vi "Periodic Tasks.vi"(8 "error in":errorcluster) -> ()   [LabVIEW 2018]
doc: "This VI runs in parallel to other tasks. It can contain as many user-defined periodic loops as you need. These can carry out PID or other sorts of timed response."
uses:
  <vilib>/Rock Robotics/WPI/Solenoid/WPI_SolenoidValue.ctl
  <vilib>/Rock Robotics/WPI/ThirdParty/Phoenix-LabVIEW/Motor Controller/Controls/CTRE_Phoenix_MotorControl_ControlMode.ctl
  <vilib>/Rock Robotics/WPI/Utilities/WPI_GetSetVariantRefNum.vi
  <vilib>/Rock Robotics/WPI/Solenoid/WPI_SolenoidSetEnum.vi
  Global 1.vi
  <vilib>/Rock Robotics/Network Tables/NT Write Boolean.vi
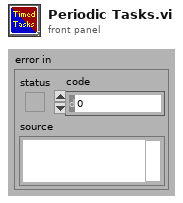
[diagram p1: front panel]
types:
  T1 = typedef "WPI_JoystickDevRef.ctl" = cluster{"Device":T2}
  T2 = typedef "WPI_JoystickDeviceEnum.ctl" = enum16{"USB 0", "USB 1", "USB 2", "USB 3", "USB 4", "USB 5"}
  T3 = typedef "WPI_RobotDriveDevRef.ctl" = cluster{"DevStatus":errorcluster, "Motors[]":T4[], "Square Inputs":bool, "Max Output":dbl}
  T4 = typedef "WPI_MotorControlDeviceRef.ctl" = cluster{"DeviceStatus":errorcluster, "Type":T5, "PWM":cluster{"PWM Channel":T6, "DeadBand":T7}, "CAN":cluster{"Device Number":u8, "SetOutput VI Ref":variant, "GetOutput VI Ref":variant, "Enable VI Ref":variant, "Disable VI Ref":variant, "Data":variant}, "Invert":bool, "DIO PWM":cluster{"PWM \"Enable\" Channel":T6, "DIOChannel":T8, "PWM Rate":dbl}}
  T5 = typedef "WPI_MotorControlType.ctl" = enum16{"PWM", "CAN", "DIO PWM"}
  T6 = typedef "FPGA_DIOPWMChannel.ctl" = enum8{"PWM 0", "PWM 1", "PWM 2", "PWM 3", "PWM 4", "PWM 5", "PWM 6", "PWM 7", "PWM 8", "PWM 9", "PWM MXP 0", "PWM MXP 1", "PWM MXP 2", "PWM MXP 3", "PWM MXP 4", "PWM MXP 5", "PWM MXP 6", "PWM MXP 7", "PWM MXP 8", "PWM MXP 9", "Invalid"}
  T7 = typedef "WPI_PWMDeadband.ctl" = cluster{"Name":string, "maxPositivePwm":i32, "minPositivePwm":i32, "centerPwm":i32, "maxNegativePwm":i32, "minNegativePwm":i32, "angularRange":u16}
  T8 = typedef "FPGA_DIOChannel.ctl" = enum8{"DIO 0", "DIO 1", "DIO 2", "DIO 3", "DIO 4", "DIO 5", "DIO 6", "DIO 7", "DIO 8", "DIO 9", "DIO MXP 0", "DIO MXP 1", "DIO MXP 2", "DIO MXP 3", "DIO MXP 4", "DIO MXP 5", "DIO MXP 6", "DIO MXP 7", "DIO MXP 8", "DIO MXP 9", "DIO MXP 10", "DIO MXP 11", "DIO MXP 12", "DIO MXP 13", "DIO MXP 14", "DIO MXP 15", "SPI Port CS1", "SPI Port CS2", "SPI Port CS3", "SPI Port MISO", "SPI Port MOSI", "Invalid"}
  T9 = cluster{"JoystickDevRef":T1, "RobotDriveDevRef":T3}
  T10 = typedef "WPI_SolenoidDevRef.ctl" = cluster{"DevStatus":errorcluster, "Pneumatics Control Module":u8, "Forward Solenoid Channel":T11, "Reverse Solenoid Channel":T11}
  T11 = typedef "WPI_SolenoidChannel.ctl" = enum8{"Solenoid 0", "Solenoid 1", "Solenoid 2", "Solenoid 3", "Solenoid 4", "Solenoid 5", "Solenoid 6", "Solenoid 7", "Invalid"}
  T12 = typedef "WPI_SolenoidValue.ctl" = enum16{"Off", "On", "Forward", "Reverse"}
  T13 = typedef "WPI_SwitchDevRef.ctl" = cluster{"DevStatus":errorcluster, "DIO Channel":T8, "CntIndex":T14, "Normally Closed":bool}
  T14 = typedef "FPGA_CounterCtrSystemIndex.ctl" = enum8{"Ctr 0", "Ctr 1", "Ctr 2", "Ctr 3", "Ctr 4", "Ctr 5", "Ctr 6", "Ctr 7", "Invalid"}
  T15 = typedef "WPI_EncoderDevRef.ctl" = cluster{"DevStatus":errorcluster, "EncoderIndex":T16, "CounterIndex":T14, "DistancePerCount":dbl, "Decoding Type":T17}
  T16 = typedef "FPGA_EncoderIdx.ctl" = enum8{"Enc 0", "Enc 1", "Enc 2", "Enc 3", "Enc 4", "Enc 5", "Enc 6", "Enc 7", "Invalid"}
  T17 = typedef "WPI_EncoderType.ctl" = enum16{"1x", "2x", "4x"}
  T18 = typedef "CTRE_Phoenix_MotorControl_ControlMode.ctl" = u16
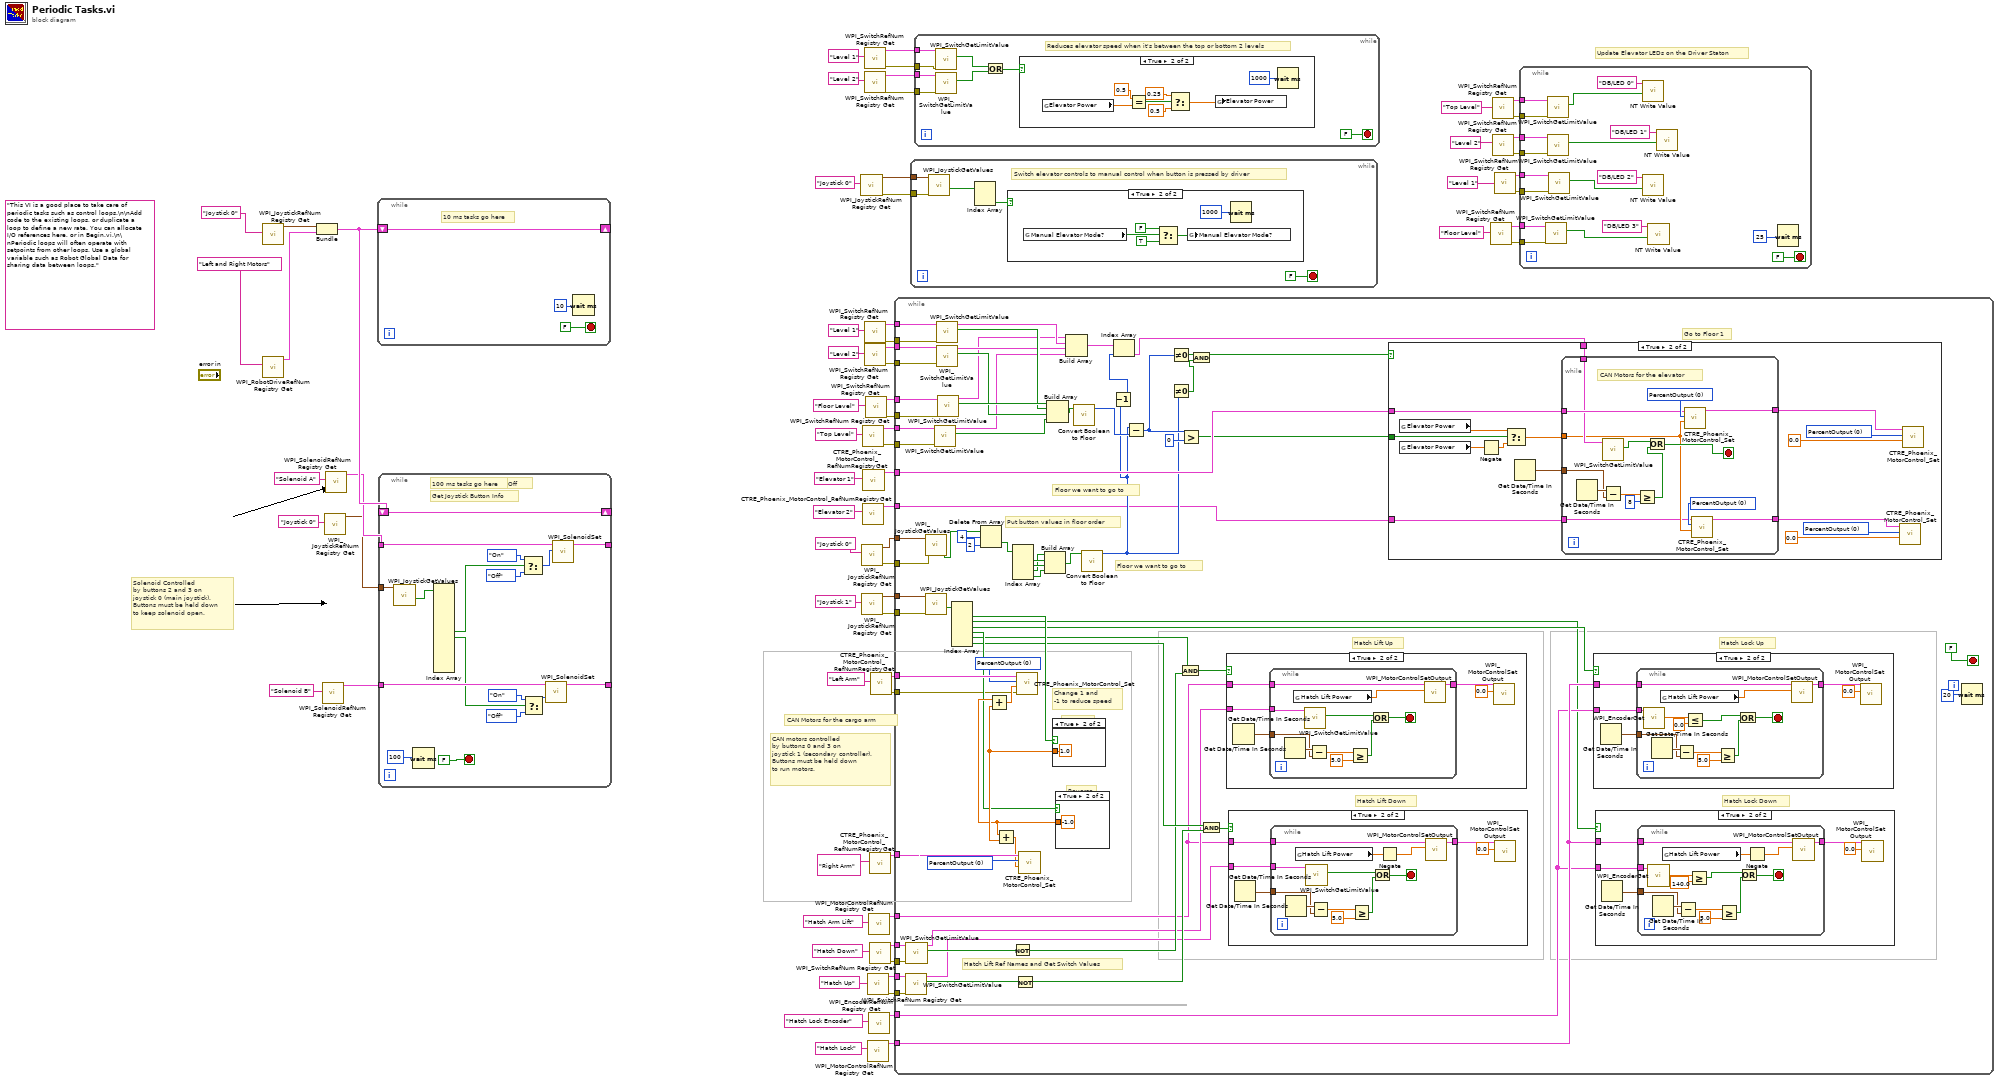
[diagram p0: block diagram]
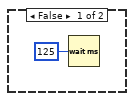
[diagram p2: hidden frame]
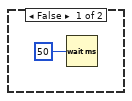
[diagram p3: hidden frame]
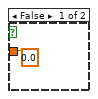
[diagram p9: hidden frame]
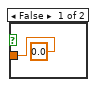
[diagram p10: hidden frame]
diagram:
  (unwired) "This VI is a good place to take care of periodic tasks such as control loops.\n\nAdd code to the existing loops, or duplicate a loop to define a new rate. You can allocate I/O references here, or in Begin.vi.\n\nPeriodic loops will often operate with setpoints from other loops. Use a global variable such as Robot Global Data for sharing data between loops."
  # "Update Elevator LEDs on the Driver Staton"
  # "CAN Motors for the cargo arm"
  # "CAN motors controlled\nby buttons 0 and 3 on \njoystick 1 (secondary controller).\nButtons must be held down\nto run motors."
  # "Solenoid Controlled\nby buttons 2 and 3 on \njoystick 0 (main joystick).\nButtons must be held down\nto keep solenoid open."
  n1 = call <vilib>:"WPI_JoystickRefNum Registry Get.vi"("refnum name"="Joystick 0") -> ("JoystickDevRef"=w69:T1)  [unwired: 1 in, 9 out]
  n2 = call <vilib>:"WPI_RobotDriveRefNum Registry Get.vi"("refnum name"="Left and Right Motors") -> ("RobotDriveDevRef"=w68:T3)  [unwired: 1 in, 9 out]
  n3 = Bundle("JoystickDevRef"=w69, "RobotDriveDevRef"=w68) -> (w67:T9)  [unwired: 1 out]
  n4 = call <vilib>:"WPI_SolenoidRefNum Registry Get.vi"("refnum name"="Solenoid B") -> ("SolenoidDevRef"=w62:T10)  [unwired: 9 in, 1 out]
  n5 = call <vilib>:"WPI_JoystickRefNum Registry Get.vi"("refnum name"="Joystick 0") -> ("JoystickDevRef"=w59:T1)  [unwired: 9 in, 1 out]
  n6 = call <vilib>:"WPI_SolenoidRefNum Registry Get.vi"("refnum name"="Solenoid A") -> ("SolenoidDevRef"=w63:T10)  [unwired: 9 in, 1 out]
  n7 = while {
    shift-right: [w72] -> _
    shift-left: w67 -> [w72]
    stop <- FALSE stop-if-true
    # "10 ms tasks go here"
    n8 = Wait (ms)(milliseconds to wait=u32 10) -> ()  [unwired: 1 out]
  }
  n9 = while {
    shift-right: [w89] -> _
    shift-left: w67 -> [w89]
    tunnel: w63 -> [w82]
    tunnel: w62 -> [w81]
    tunnel: [w80] -> _
    tunnel: [w79] -> _
    tunnel: w59 -> [w78]
    stop <- FALSE stop-if-true
    # "Get Joystick Button Info"
    # "Turn the solenoid On or Off"
    # "100 ms tasks go here"
    n10 = call <vilib>:"WPI_JoystickGetValues.vi"("JoystickDevRef"=w78) -> ("Buttons"=w77:bool[])  [unwired: 6 in, 4 out]
    n11 = Wait (ms)(milliseconds to wait=u32 100) -> ()  [unwired: 1 out]
    n12 = Index Array(array=w77) -> (element #7=w76:bool, element #8=w75:bool)  [unwired: 14 in, 12 out]
    n13 = Select(t=WPI_SolenoidValue."On" ("Value"), s=w76, f=WPI_SolenoidValue."Off" ("Value")) -> (s? t:f=w86:T12)
    n14 = Select(t=WPI_SolenoidValue."On" ("Value"), s=w75, f=WPI_SolenoidValue."Off" ("Value")) -> (s? t:f=w83:T12)
    n15 = call-poly <vilib>:"WPI_SolenoidSet.vi"("Value"=w83, "SolenoidDevRef"=w81) -> ("SolenoidDevRef"=w79:T10)  [unwired: 1 in, 8 out]
    n16 = call-poly <vilib>:"WPI_SolenoidSet.vi"("Value"=w86, "SolenoidDevRef"=w82) -> ("SolenoidDevRef"=w80:T10)  [unwired: 1 in, 8 out]
  }
  n17 = call <vilib>:"WPI_JoystickRefNum Registry Get.vi"("refnum name"="Joystick 0") -> ("error out"=w46:errorcluster, "JoystickDevRef"=w47:T1)  [unwired: 9 in]
  n18 = call <vilib>:"WPI_JoystickRefNum Registry Get.vi"("refnum name"="Joystick 0") -> ("error out"=w40:errorcluster, "JoystickDevRef"=w53:T1)  [unwired: 9 in]
  n19 = call <vilib>:"WPI_JoystickRefNum Registry Get.vi"("refnum name"="Joystick 1") -> ("error out"=w45:errorcluster, "JoystickDevRef"=w55:T1)  [unwired: 9 in]
  n20 = call <vilib>:"WPI_SwitchRefNum Registry Get.vi"("refnum name"="Top Level") -> ("error out"=w44:errorcluster, "SwitchDevRef"=w56:T13)  [unwired: 9 in]
  n21 = call <vilib>:"CTRE_Phoenix_MotorControl_RefNumRegistryGet.vi"("refnum name"="Elevator 2") -> ("PhoenixMotorControlDevRef"=w7:T4)  [unwired: 9 in, 1 out]
  n22 = call <vilib>:"CTRE_Phoenix_MotorControl_RefNumRegistryGet.vi"("refnum name"="Elevator 1") -> ("PhoenixMotorControlDevRef"=w54:T4)  [unwired: 9 in, 1 out]
  n23 = call <vilib>:"WPI_SwitchRefNum Registry Get.vi"("refnum name"="Level 1") -> ("error out"=w1:errorcluster, "SwitchDevRef"=w4:T13)  [unwired: 9 in]
  n24 = call <vilib>:"WPI_SwitchRefNum Registry Get.vi"("refnum name"="Level 2") -> ("error out"=w2:errorcluster, "SwitchDevRef"=w3:T13)  [unwired: 9 in]
  n25 = call <vilib>:"WPI_SwitchRefNum Registry Get.vi"("refnum name"="Level 1") -> ("error out"=w41:errorcluster, "SwitchDevRef"=w66:T13)  [unwired: 9 in]
  n26 = call <vilib>:"WPI_SwitchRefNum Registry Get.vi"("refnum name"="Level 2") -> ("error out"=w42:errorcluster, "SwitchDevRef"=w65:T13)  [unwired: 9 in]
  n27 = call <vilib>:"WPI_SwitchRefNum Registry Get.vi"("refnum name"="Floor Level") -> ("error out"=w43:errorcluster, "SwitchDevRef"=w52:T13)  [unwired: 9 in]
  n28 = call <vilib>:"WPI_SwitchRefNum Registry Get.vi"("refnum name"="Hatch Up") -> ("error out"=w22:errorcluster, "SwitchDevRef"=w23:T13)  [unwired: 9 in]
  n29 = call <vilib>:"WPI_MotorControlRefNum Registry Get.vi"("refnum name"="Hatch Lock") -> ("MotorControlDevRef"=w17:T4)  [unwired: 9 in, 1 out]
  n30 = call <vilib>:"WPI_MotorControlRefNum Registry Get.vi"("refnum name"="Hatch Arm Lift") -> ("MotorControlDevRef"=w19:T4)  [unwired: 9 in, 1 out]
  n31 = call <vilib>:"WPI_EncoderRefNum Registry Get.vi"("refnum name"="Hatch Lock Encoder") -> ("EncoderDevRef"=w18:T15)  [unwired: 9 in, 1 out]
  n32 = call <vilib>:"WPI_SwitchRefNum Registry Get.vi"("refnum name"="Hatch Down") -> ("error out"=w21:errorcluster, "SwitchDevRef"=w20:T13)  [unwired: 9 in]
  n33 = call <vilib>:"CTRE_Phoenix_MotorControl_RefNumRegistryGet.vi"("refnum name"="Right Arm") -> ("PhoenixMotorControlDevRef"=w57:T4)  [unwired: 9 in, 1 out]
  n34 = call <vilib>:"CTRE_Phoenix_MotorControl_RefNumRegistryGet.vi"("refnum name"="Left Arm") -> ("error out"=w39:errorcluster, "PhoenixMotorControlDevRef"=w58:T4)  [unwired: 9 in]
  n35 = while {
    tunnel: w66 -> [w165]
    tunnel: w65 -> [w164]
    tunnel: w58 -> [w163]
    tunnel: w57 -> [w162]
    tunnel: w56 -> [w161]
    tunnel: w55 -> [w160]
    tunnel: w54 -> [w157]
    tunnel: w53 -> [w159]
    tunnel: w52 -> [w158]
    tunnel: w45 -> [w147]
    tunnel: w44 -> [w146]
    tunnel: w43 -> [w145]
    tunnel: w42 -> [w144]
    tunnel: w41 -> [w143]
    tunnel: w40 -> [w142]
    tunnel: w39 -> [w141]
    tunnel: w23 -> [w140]
    tunnel: w22 -> [w139]
    tunnel: w21 -> [w138]
    tunnel: w20 -> [w137]
    tunnel: w19 -> [w127]
    tunnel: w18 -> [w124]
    tunnel: w17 -> [w125]
    tunnel: w7 -> [w92]
    stop <- FALSE stop-if-true
    w154 = T18 0 items=["PercentOutput"=0, "Position"=1, "Velocity"=2, "Current"=3, "Follower"=5, "MotionProfile"=6, "MotionMagic"=7, "MotionProfileArc"=10, "Disabled"=15] ("Control Mode")
    w156 = T18 0 items=["PercentOutput"=0, "Position"=1, "Velocity"=2, "Current"=3, "Follower"=5, "MotionProfile"=6, "MotionMagic"=7, "MotionProfileArc"=10, "Disabled"=15] ("Control Mode")
    # "Put button values in floor order"
    # "Floor we want to go to"
    # "Floor we want to go to"
    # "Go to Floor 1"
    # "Hatch Lock Down"
    # "Hatch Lock Up"
    # "Hatch Lift Ref Names and Get Switch Values"
    # "Hatch Lift Down"
    # "Hatch Lift Up"
    # "Change 1 and\n-1 to reduce speed"
    # "Forward"
    # "Reverse"
    n36 = call <vilib>:"WPI_SwitchGetLimitValue.vi"("error in (no error)"=w139, "SwitchDevRef"=w140) -> ("Switch Pressed"=w134:bool, "SwitchDevRef"=w126:T13)  [unwired: 7 in, 1 out]
    n37 = call <vilib>:"WPI_SwitchGetLimitValue.vi"("error in (no error)"=w138, "SwitchDevRef"=w137) -> ("Switch Pressed"=w132:bool, "SwitchDevRef"=w128:T13)  [unwired: 7 in, 1 out]
    n38 = call <vilib>:"WPI_JoystickGetValues.vi"("error in (no error)"=w142, "JoystickDevRef"=w159) -> ("Buttons"=w93:bool[])  [unwired: 5 in, 4 out]
    n39 = call <vilib>:"WPI_JoystickGetValues.vi"("error in (no error)"=w147, "JoystickDevRef"=w160) -> ("Buttons"=w151:bool[])  [unwired: 5 in, 4 out]
    n40 = call <vilib>:"WPI_SwitchGetLimitValue.vi"("error in (no error)"=w146, "SwitchDevRef"=w161) -> ("Switch Pressed"=w118:bool, "SwitchDevRef"=w101:T13)  [unwired: 7 in, 1 out]
    n41 = call <vilib>:"WPI_SwitchGetLimitValue.vi"("error in (no error)"=w143, "SwitchDevRef"=w165) -> ("Switch Pressed"=w110:bool, "SwitchDevRef"=w103:T13)  [unwired: 7 in, 1 out]
    n42 = call <vilib>:"WPI_SwitchGetLimitValue.vi"("error in (no error)"=w144, "SwitchDevRef"=w164) -> ("Switch Pressed"=w109:bool, "SwitchDevRef"=w102:T13)  [unwired: 7 in, 1 out]
    n43 = call <vilib>:"WPI_SwitchGetLimitValue.vi"("error in (no error)"=w145, "SwitchDevRef"=w158) -> ("Switch Pressed"=w117:bool, "SwitchDevRef"=w100:T13)  [unwired: 7 in, 1 out]
    n44 = Index Array(array=w151) -> (element #1=w149:bool, element #2=w122:bool, element #3=w123:bool, element #4=w148:bool, element #5=w136:bool, element #6=w135:bool)  [unwired: 6 in]
    n45 = Delete From Array(array=w93, length=4, index=2) -> (deleted portion=w116:bool[])  [unwired: 1 out]
    n46 = Not(x=w132) -> (.not. x?=w131:bool)
    n47 = Index Array(array=w116) -> (element #1=w115:bool, element #2=w114:bool, element #3=w113:bool, element #4=w112:bool)  [unwired: 4 in]
    n48 = Not(x=w134) -> (.not. x?=w130:bool)
    n49 = Build Array(w113, w115, w114, w112) -> (w111:bool[])
    n50 = Build Array(w117, w110, w109, w118) -> (w119:bool[])
    n51 = case shown="True" w149 {
      tunnel: [0.0 1.0] -> w152
      frame False {
      }
      frame True {
      }
    }
    n52 = case shown="True" w148 {
      tunnel: [0.0 -1.0] -> w150
      frame False {
      }
      frame True {
      }
    }
    n53 = Add(x=w150, y=w152) -> (x+y=w155:dbl)
    n54 = Add(x=w150, y=w152) -> (x+y=w153:dbl)
    n55 = call <vilib>:"CTRE_Phoenix_MotorControl_Set.vi"("error in (no error)"=w141, "Output"=w155, "Control Mode"=w156, "PhoenixMotorControlDevRef"=w163) -> ()  [unwired: 6 in, 2 out]
    n56 = call <vilib>:"CTRE_Phoenix_MotorControl_Set.vi"("Output"=w153, "Control Mode"=w154, "PhoenixMotorControlDevRef"=w162) -> ()  [unwired: 7 in, 2 out]
    n57 = Build Array(w100, w103, w102, w101) -> (w99:T13[])
    n58 = call "Convert Boolean to Floor.vi"("Boolean array"=w119) -> ("Floor Number"=w107:i32)  [unwired: 8 in, 2 out]
    n59 = call "Convert Boolean to Floor.vi"("Boolean array"=w111) -> ("Floor Number"=w95:i32)  [unwired: 8 in, 2 out]
    n60 = Decrement(x=w95) -> (x-1=w97:i32)
    n61 = Index Array(array=w99, index=w97) -> (element=w98:T13)
    n62 = Subtract(x=w95, y=w107) -> (x-y=w106:i32)
    n63 = Not Equal To 0?(x=w106) -> (x != 0?=w108:bool)
    n64 = Not Equal To 0?(x=w95) -> (x != 0?=w94:bool)
    n65 = And(x=w136, y=w131) -> (x .and. y?=w133:bool)
    n66 = Greater?(x=w106, y=0) -> (0:w104:bool)
    n67 = And(x=w108, y=w94) -> (x .and. y?=w96:bool)
    n68 = And(x=w135, y=w130) -> (x .and. y?=w129:bool)
    n69 = case shown="True" w133 {
      tunnel: w128 -> [_ w256]
      tunnel: w127 -> [_ w255]
      frame False {
      }
      frame True {
        n70 = Get Date/Time In Seconds() -> (seconds since 1Jan1904=w254:timestamp)
        n71 = while {
          tunnel: w256 -> [w267]
          tunnel: w255 -> [w266]
          tunnel: w254 -> [w262]
          tunnel: [w258] -> w253
          stop <- w261 stop-if-true
          n72 = Get Date/Time In Seconds() -> (seconds since 1Jan1904=w263:timestamp)
          n73 = global read "Global 1.vi" "Hatch Lift Power"() -> (w265:dbl)
          n74 = call <vilib>:"WPI_SwitchGetLimitValue.vi"("SwitchDevRef"=w267) -> ("Switch Pressed"=w260:bool)  [unwired: 8 in, 2 out]
          n75 = Subtract(x=w263, y=w262) -> (x-y=w264:dbl)
          n76 = Greater Or Equal?(x=w264, y=5.0) -> (x >= y?=w259:bool)
          n77 = Or(x=w260, y=w259) -> (x .or. y?=w261:bool)
          n78 = call <vilib>:"WPI_MotorControlSetOutput.vi"("Output"=w265, "MotorControlDevRef"=w266) -> ("MotorControlDevRef"=w258:T4)  [unwired: 7 in, 2 out]
        }
        n79 = call <vilib>:"WPI_MotorControlSetOutput.vi"("Output"=0.0, "MotorControlDevRef"=w253) -> ()  [unwired: 7 in, 3 out]
      }
    }
    n80 = case shown="True" w129 {
      tunnel: w126 -> [_ w239]
      tunnel: w127 -> [_ w238]
      frame False {
      }
      frame True {
        n81 = Get Date/Time In Seconds() -> (seconds since 1Jan1904=w237:timestamp)
        n82 = while {
          tunnel: w239 -> [w251]
          tunnel: w238 -> [w250]
          tunnel: w237 -> [w246]
          tunnel: [w242] -> w236
          stop <- w245 stop-if-true
          n83 = Get Date/Time In Seconds() -> (seconds since 1Jan1904=w247:timestamp)
          n84 = global read "Global 1.vi" "Hatch Lift Power"() -> (w249:dbl)
          n85 = call <vilib>:"WPI_SwitchGetLimitValue.vi"("SwitchDevRef"=w251) -> ("Switch Pressed"=w244:bool)  [unwired: 8 in, 2 out]
          n86 = Subtract(x=w247, y=w246) -> (x-y=w248:dbl)
          n87 = Greater Or Equal?(x=w248, y=5.0) -> (x >= y?=w243:bool)
          n88 = Or(x=w244, y=w243) -> (x .or. y?=w245:bool)
          n89 = Negate(x=w249) -> (-x=w241:dbl)
          n90 = call <vilib>:"WPI_MotorControlSetOutput.vi"("Output"=w241, "MotorControlDevRef"=w250) -> ("MotorControlDevRef"=w242:T4)  [unwired: 7 in, 2 out]
        }
        n91 = call <vilib>:"WPI_MotorControlSetOutput.vi"("Output"=0.0, "MotorControlDevRef"=w236) -> ()  [unwired: 7 in, 3 out]
      }
    }
    n92 = case shown="True" w96 {
      tunnel: w157 -> [_ w182]
      tunnel: w98 -> [_ w178]
      tunnel: w104 -> [_ w175]
      tunnel: w92 -> [_ w168]
      frame False {
      }
      frame True {
        w171 = T18 0 items=["PercentOutput"=0, "Position"=1, "Velocity"=2, "Current"=3, "Follower"=5, "MotionProfile"=6, "MotionMagic"=7, "MotionProfileArc"=10, "Disabled"=15] ("Control Mode")
        w181 = T18 0 items=["PercentOutput"=0, "Position"=1, "Velocity"=2, "Current"=3, "Follower"=5, "MotionProfile"=6, "MotionMagic"=7, "MotionProfileArc"=10, "Disabled"=15] ("Control Mode")
        n93 = global read "Global 1.vi" "Elevator Power"() -> (w174:dbl)
        n94 = global read "Global 1.vi" "Elevator Power"() -> (w172:dbl)
        n95 = Negate(x=w172) -> (-x=w173:dbl)
        n96 = Select(t=w174, s=w175, f=w173) -> (s? t:f=w177:dbl)
        n97 = Get Date/Time In Seconds() -> (seconds since 1Jan1904=w176:timestamp)
        n98 = while {
          tunnel: w182 -> [w196]
          tunnel: [w195] -> w179
          tunnel: w178 -> [w194]
          tunnel: w177 -> [w186]
          tunnel: w176 -> [w190]
          tunnel: [w184] -> w170
          tunnel: w168 -> [w183]
          stop <- w193 stop-if-true
          w185 = T18 0 items=["PercentOutput"=0, "Position"=1, "Velocity"=2, "Current"=3, "Follower"=5, "MotionProfile"=6, "MotionMagic"=7, "MotionProfileArc"=10, "Disabled"=15] ("Control Mode")
          w197 = T18 0 items=["PercentOutput"=0, "Position"=1, "Velocity"=2, "Current"=3, "Follower"=5, "MotionProfile"=6, "MotionMagic"=7, "MotionProfileArc"=10, "Disabled"=15] ("Control Mode")
          # "CAN Motors for the elevator"
          n99 = Get Date/Time In Seconds() -> (seconds since 1Jan1904=w191:timestamp)
          n100 = call <vilib>:"WPI_SwitchGetLimitValue.vi"("SwitchDevRef"=w194) -> ("Switch Pressed"=w192:bool)  [unwired: 8 in, 2 out]
          n101 = Subtract(x=w191, y=w190) -> (x-y=w188:dbl)
          n102 = Greater Or Equal?(x=w188, y=8) -> (x >= y?=w187:bool)
          n103 = Or(x=w192, y=w187) -> (x .or. y?=w193:bool)
          n104 = call <vilib>:"CTRE_Phoenix_MotorControl_Set.vi"("Output"=w186, "Control Mode"=w197, "PhoenixMotorControlDevRef"=w196) -> ("PhoenixMotorControlDevRef"=w195:T4)  [unwired: 7 in, 1 out]
          n105 = call <vilib>:"CTRE_Phoenix_MotorControl_Set.vi"("Output"=w186, "Control Mode"=w185, "PhoenixMotorControlDevRef"=w183) -> ("PhoenixMotorControlDevRef"=w184:T4)  [unwired: 7 in, 1 out]
        }
        n106 = call <vilib>:"CTRE_Phoenix_MotorControl_Set.vi"("Output"=0.0, "Control Mode"=w171, "PhoenixMotorControlDevRef"=w170) -> ()  [unwired: 7 in, 2 out]
        n107 = call <vilib>:"CTRE_Phoenix_MotorControl_Set.vi"("Output"=0.0, "Control Mode"=w181, "PhoenixMotorControlDevRef"=w179) -> ()  [unwired: 7 in, 2 out]
      }
    }
    n108 = case shown="True" w123 {
      tunnel: w125 -> [_ w221]
      tunnel: w124 -> [_ w217]
      frame False {
      }
      frame True {
        n109 = Get Date/Time In Seconds() -> (seconds since 1Jan1904=w220:timestamp)
        n110 = while {
          tunnel: w221 -> [w234]
          tunnel: w220 -> [w230]
          tunnel: [w227] -> w219
          tunnel: w217 -> [w222]
          stop <- w229 stop-if-true
          n111 = call <vilib>:"WPI_EncoderGet.vi"("EncoderDevRef"=w222) -> ("Distance"=w225:dbl)  [unwired: 5 in, 5 out]
          n112 = Get Date/Time In Seconds() -> (seconds since 1Jan1904=w231:timestamp)
          n113 = global read "Global 1.vi" "Hatch Lift Power"() -> (w233:dbl)
          n114 = Subtract(x=w231, y=w230) -> (x-y=w232:dbl)
          n115 = Less Or Equal?(x=w225, y=0.0) -> (x <= y?=w223:bool)
          n116 = Greater Or Equal?(x=w232, y=5.0) -> (x >= y?=w228:bool)
          n117 = Or(x=w223, y=w228) -> (x .or. y?=w229:bool)
          n118 = call <vilib>:"WPI_MotorControlSetOutput.vi"("Output"=w233, "MotorControlDevRef"=w234) -> ("MotorControlDevRef"=w227:T4)  [unwired: 7 in, 2 out]
        }
        n119 = call <vilib>:"WPI_MotorControlSetOutput.vi"("Output"=0.0, "MotorControlDevRef"=w219) -> ()  [unwired: 7 in, 3 out]
      }
    }
    n120 = case shown="True" w122 {
      tunnel: w125 -> [_ w202]
      tunnel: w124 -> [_ w198]
      frame False {
      }
      frame True {
        n121 = Get Date/Time In Seconds() -> (seconds since 1Jan1904=w201:timestamp)
        n122 = while {
          tunnel: w202 -> [w216]
          tunnel: w201 -> [w212]
          tunnel: [w209] -> w200
          tunnel: w198 -> [w206]
          stop <- w211 stop-if-true
          n123 = call <vilib>:"WPI_EncoderGet.vi"("EncoderDevRef"=w206) -> ("Distance"=w205:dbl)  [unwired: 5 in, 5 out]
          n124 = Get Date/Time In Seconds() -> (seconds since 1Jan1904=w213:timestamp)
          n125 = global read "Global 1.vi" "Hatch Lift Power"() -> (w215:dbl)
          n126 = Subtract(x=w213, y=w212) -> (x-y=w214:dbl)
          n127 = Greater Or Equal?(x=w205, y=140.0) -> (x >= y?=w204:bool)
          n128 = Greater Or Equal?(x=w214, y=5.0) -> (x >= y?=w210:bool)
          n129 = Or(x=w204, y=w210) -> (x .or. y?=w211:bool)
          n130 = Negate(x=w215) -> (-x=w208:dbl)
          n131 = call <vilib>:"WPI_MotorControlSetOutput.vi"("Output"=w208, "MotorControlDevRef"=w216) -> ("MotorControlDevRef"=w209:T4)  [unwired: 7 in, 2 out]
        }
        n132 = call <vilib>:"WPI_MotorControlSetOutput.vi"("Output"=0.0, "MotorControlDevRef"=w200) -> ()  [unwired: 7 in, 3 out]
      }
    }
    n133 = Wait (ms)(milliseconds to wait=u32 20) -> ()  [unwired: 1 out]
  }
  n134 = while {
    tunnel: w47 -> [w276]
    tunnel: w46 -> [w275]
    stop <- FALSE stop-if-true
    # "Switch elevator controls to manual control when button is pressed by driver"
    n135 = call <vilib>:"WPI_JoystickGetValues.vi"("error in (no error)"=w275, "JoystickDevRef"=w276) -> ("Buttons"=w274:bool[])  [unwired: 5 in, 4 out]
    n136 = Index Array(array=w274) -> (element #2=w273:bool)  [unwired: 2 in, 1 out]
    n137 = case shown="True" w273 {
      frame False {
        n138 = Wait (ms)(milliseconds to wait=u32 50) -> ()  [unwired: 1 out]
      }
      frame True {
        n139 = global read "Global 1.vi" "Manual Elevator Mode?"() -> (w282:bool)
        n140 = Select(t=FALSE, s=w282, f=TRUE) -> (s? t:f=w281:bool)
        n141 = global write "Global 1.vi" "Manual Elevator Mode?"(w281) -> ()
        n142 = Wait (ms)(milliseconds to wait=u32 1000) -> ()  [unwired: 1 out]
      }
    }
  }
  n143 = while {
    tunnel: w4 -> [w290]
    tunnel: w3 -> [w289]
    tunnel: w2 -> [w288]
    tunnel: w1 -> [w287]
    stop <- FALSE stop-if-true
    # "Reduces elevator speed when it's between the top or bottom 2 levels"
    n144 = call <vilib>:"WPI_SwitchGetLimitValue.vi"("error in (no error)"=w287, "SwitchDevRef"=w290) -> ("Switch Pressed"=w286:bool)  [unwired: 7 in, 2 out]
    n145 = call <vilib>:"WPI_SwitchGetLimitValue.vi"("error in (no error)"=w288, "SwitchDevRef"=w289) -> ("Switch Pressed"=w284:bool)  [unwired: 7 in, 2 out]
    n146 = Or(x=w286, y=w284) -> (x .or. y?=w285:bool)
    n147 = case shown="True" w285 {
      frame False {
        n148 = Wait (ms)(milliseconds to wait=u32 125) -> ()  [unwired: 1 out]
      }
      frame True {
        n149 = global read "Global 1.vi" "Elevator Power"() -> (w298:dbl)
        n150 = Equal?(x=0.5, y=w298) -> (x = y?=w297:bool)
        n151 = Select(t=0.25, s=w297, f=0.5) -> (s? t:f=w293:dbl)
        n152 = global write "Global 1.vi" "Elevator Power"(w293) -> ()
        n153 = Wait (ms)(milliseconds to wait=u32 1000) -> ()  [unwired: 1 out]
      }
    }
  }
  n154 = call <vilib>:"WPI_SwitchRefNum Registry Get.vi"("refnum name"="Floor Level") -> ("error out"=w33:errorcluster, "SwitchDevRef"=w32:T13)  [unwired: 9 in]
  n155 = call <vilib>:"WPI_SwitchRefNum Registry Get.vi"("refnum name"="Top Level") -> ("error out"=w37:errorcluster, "SwitchDevRef"=w38:T13)  [unwired: 9 in]
  n156 = call <vilib>:"WPI_SwitchRefNum Registry Get.vi"("refnum name"="Level 2") -> ("error out"=w35:errorcluster, "SwitchDevRef"=w36:T13)  [unwired: 9 in]
  n157 = call <vilib>:"WPI_SwitchRefNum Registry Get.vi"("refnum name"="Level 1") -> ("error out"=w31:errorcluster, "SwitchDevRef"=w34:T13)  [unwired: 9 in]
  n158 = while {
    tunnel: w38 -> [w316]
    tunnel: w37 -> [w315]
    tunnel: w36 -> [w314]
    tunnel: w35 -> [w313]
    tunnel: w34 -> [w312]
    tunnel: w33 -> [w311]
    tunnel: w32 -> [w310]
    tunnel: w31 -> [w309]
    stop <- FALSE stop-if-true
    n159 = call <vilib>:"WPI_SwitchGetLimitValue.vi"("error in (no error)"=w311, "SwitchDevRef"=w310) -> ("Switch Pressed"=w301:bool)  [unwired: 7 in, 2 out]
    n160 = call <vilib>:"WPI_SwitchGetLimitValue.vi"("error in (no error)"=w315, "SwitchDevRef"=w316) -> ("Switch Pressed"=w307:bool)  [unwired: 7 in, 2 out]
    n161 = call <vilib>:"WPI_SwitchGetLimitValue.vi"("error in (no error)"=w313, "SwitchDevRef"=w314) -> ("Switch Pressed"=w305:bool)  [unwired: 7 in, 2 out]
    n162 = call <vilib>:"WPI_SwitchGetLimitValue.vi"("error in (no error)"=w309, "SwitchDevRef"=w312) -> ("Switch Pressed"=w303:bool)  [unwired: 7 in, 2 out]
    n163 = call-poly <vilib>:"NT Write Value.vi"("Boolean"=w307, "Name"="DB/LED 0") -> ()  [unwired: 9 in, 1 out]
    n164 = call-poly <vilib>:"NT Write Value.vi"("Boolean"=w303, "Name"="DB/LED 2") -> ()  [unwired: 9 in, 1 out]
    n165 = call-poly <vilib>:"NT Write Value.vi"("Boolean"=w301, "Name"="DB/LED 3") -> ()  [unwired: 9 in, 1 out]
    n166 = call-poly <vilib>:"NT Write Value.vi"("Boolean"=w305, "Name"="DB/LED 1") -> ()  [unwired: 9 in, 1 out]
    n167 = Wait (ms)(milliseconds to wait=u32 25 ("millisecond timer value")) -> ()  [unwired: 1 out]
  }
